vi "Add Text Input.vi"(7 "id":string, 8 "error in (no error)":errorcluster, 9 "Placeholder Text":string, 10 "Title":string, 11 "ToastBuilder in":refnum<class "ToastBuilder.lvclass">) -> (0 "error out":errorcluster, 3 "ToastBuilder out":refnum<class "ToastBuilder.lvclass">)   [LabVIEW 2026, in "ToastNotification.lvlib" / "ToastBuilder.lvclass"]
doc: "Add a text input to the native builder. id identifies the value returned under Activation.User Inputs.Key. Title is the visible field label; Placeholder Text is a hint displayed while the field is empty, not an initial value. Add a button to submit the reply. Call before Show. Skip on incoming error and preserve the input builder; validation is delegated to the native toolkit."
uses:
  ToastBuilder.lvclass
  ToastBuilder.lvclass/ToastBuilder.ctl
  Read Builder Reference.vi
  Write Builder Reference.vi
  Toast Native/Toast Native.lvlib
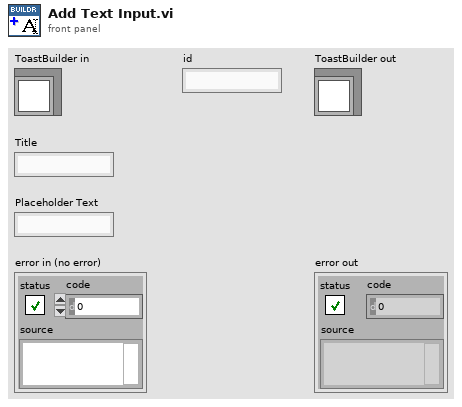
[diagram p1: front panel]
types:
  T1 = typedef "ToastNotification.lvlib/ToastBuilder.lvclass/Builder Reference.ctl" = refnum<k24>
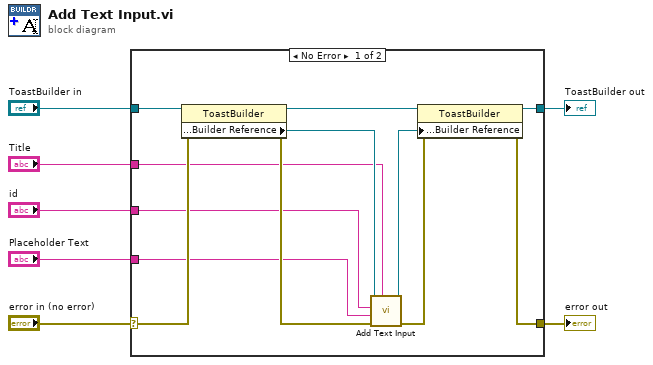
[diagram p0: block diagram]
diagram:
  n1 = case shown="No Error" "error in (no error)" {
    selector: "error in (no error)" -> [w16 w21]
    tunnel: [w15 w21] -> w6
    tunnel: [w17 w20] -> w4
    tunnel: "ToastBuilder in" -> [w19 w20]
    tunnel: "id" -> [w10 _]
    tunnel: "Placeholder Text" -> [w9 _]
    tunnel: "Title" -> [w8 _]
    frame No Error {
      n2 = property class="ToastBuilder"(reference=w19, error in=w16) -> (reference out=w18:refnum<class "ToastBuilder.lvclass">, error out=w14:errorcluster, "Public:Properties:Builder Reference"=w12:T1)
      n3 = call "Add Text Input.vi"("title"=w8, "error in (no error)"=w14, "placeHolderContent"=w9, "id"=w10, "reference"=w12) -> ("error out"=w13:errorcluster, "reference out"=w11:refnum<k24>)  [unwired: 5 in]
      n4 = property class="ToastBuilder"(reference=w18, error in=w13, "Public:Properties:Builder Reference"=w11) -> (reference out=w17:refnum<class "ToastBuilder.lvclass">, error out=w15:errorcluster)
    }
    frame Error {
    }
  }
  "error out" <- w6
  "ToastBuilder out" <- w4
